vi "Set Mode.vi"(8 "error in":errorcluster, 10 "Parameter Mode":T1, 11 "Element in":refnum<class "Element.lvclass">) -> (0 "error out":errorcluster, 3 "Element out":refnum<class "Element.lvclass">)   [LabVIEW 2026, in "Element.lvclass"]
doc: "Set Mode."
uses:
  Element.lvclass
  Type Definitions/Parameter Mode--enum.ctl
  Element.lvclass/Element.ctl
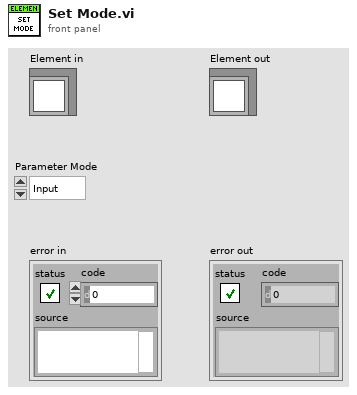
[diagram p1: front panel]
types:
  T1 = typedef "Parameter Mode--enum.ctl" = enum16{"Input", "Output"}
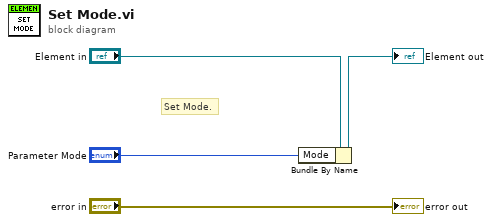
[diagram p0: block diagram]
diagram:
  # "Set Mode."
  n1 = Bundle By Name(cluster="Element in", "Mode"="Parameter Mode") -> (→"Element out":refnum<class "Element.lvclass">)
  "error out" <- "error in"
